vi "test--colorable decorations.vi"() -> ()   [LabVIEW 2021]
doc: "This VI will be used to test out the label creation and deletion, the quick drop list of controls, and the theme change"
panel:
  in  "Listbox 2":i32(listbox)
  in  "Numeric 3":dbl
  in  "Text Ring":u16(ring)
  out "Numeric 2":dbl
  in  "Numeric":dbl
  in  "Table Control":string[][](table)
  in  "Listbox":i32(listbox)
  in  "Multicolumn Listbox":i32(listbox)
  in  "String":string
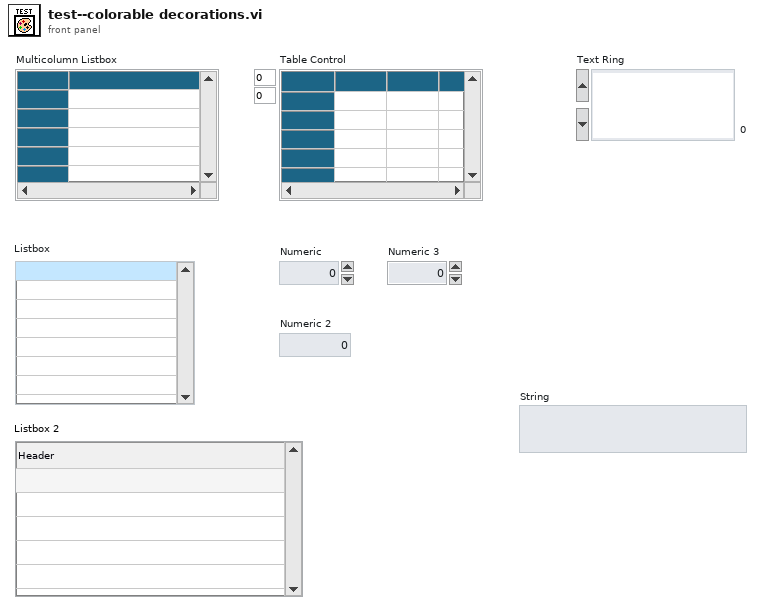
[diagram p1: front panel]
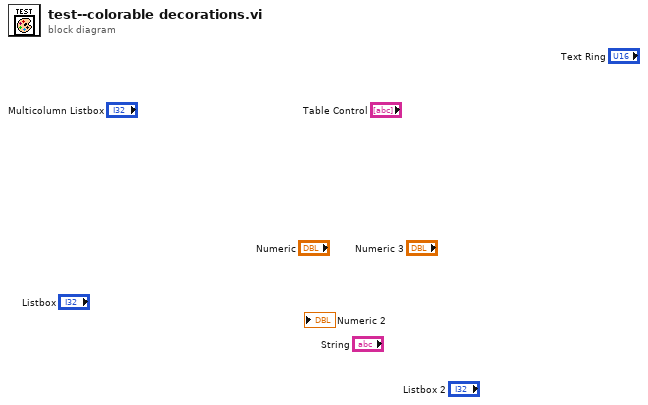
[diagram p0: block diagram]
diagram:
